vi "VIH Project - Get Effective Group Rule.vi"(7 "Ignore Control Rules (F)":bool, 8 "error in":errorcluster, 10 "Group ID":string, 11 "Project Tree":T1) -> (0 "error out":errorcluster, 2 "Effective Group Rule":T2, 3 "dup Project Tree":T1)   [LabVIEW 2014]
doc: "::: VI Helpeks :::\nCopyright (c) 2000-2026 Konstantin Shifershteyn. All rights reserved."
uses:
  VIH Project Tree Typedef - Tree Refnum.ctl
  _VIH HelpGen.llb/VIH HelpGen Typedef - Cluster - Group Rule.ctl
  _VIH HelpGen.llb/VIH HelpGen Typedef - Enum - Default,Enable,Disable.ctl
  _VIH HelpGen.llb/VIH HelpGen Typedef - Cluster - Group Rule - Source Paths.ctl
  _VIH HelpGen.llb/VIH HelpGen Typedef - Cluster - Group Rule - Target Paths.ctl
  _VIH HelpGen.llb/VIH HelpGen Typedef - Enum - Description Mode.ctl
  _VIH HelpGen.llb/VIH HelpGen Typedef - Cluster - Control Rule.ctl
  _VIH HelpGen.llb/VIH HelpGen Typedef - Cluster - Enum Value Info.ctl
  _VIH HelpGen.llb/VIH HelpGen Typedef - Cluster - Group Rule - Flags.ctl
  VIH Project Tree Typedef - Tree Item Type.ctl
panel:
  # "VI Helpeks\nCopyright (c) 2012-2026 Konstantin Shifershteyn"
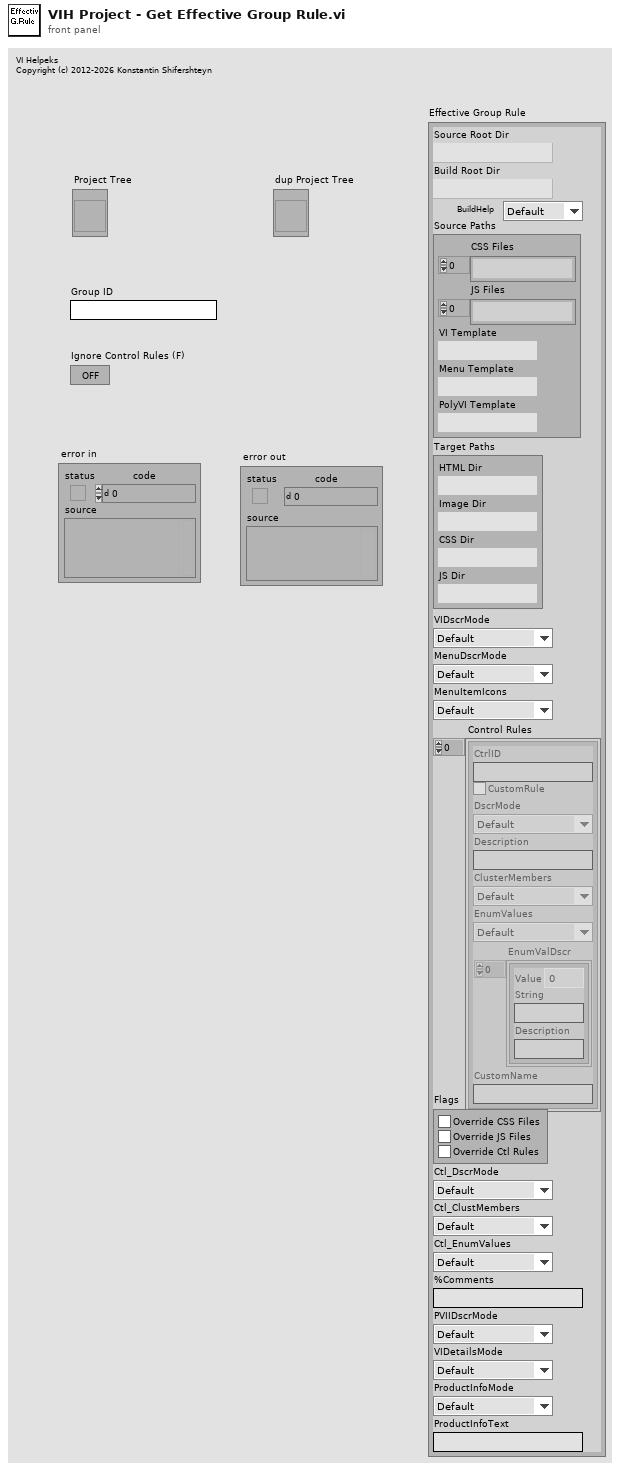
[diagram p1: front panel]
types:
  T1 = typedef "VIH Project Tree Typedef - Tree Refnum.ctl" = refnum<vi>
  T2 = typedef "VIH HelpGen Typedef - Cluster - Group Rule.ctl" = cluster{"Source Root Dir":path, "Build Root Dir":path, "BuildHelp":T3, "Source Paths":T4, "Target Paths":T5, "VIDscrMode":T6, "MenuDscrMode":T6, "MenuItemIcons":T3, "Control Rules":T7[], "Flags":T9, "Ctl_DscrMode":T6, "Ctl_ClustMembers":T3, "Ctl_EnumValues":T3, "%Comments":string, "PVIIDscrMode":T6, "VIDetailsMode":T6, "ProductInfoMode":T3, "ProductInfoText":string}
  T3 = typedef "VIH HelpGen Typedef - Enum - Default,Enable,Disable.ctl" = enum16{"Default", "Enable", "Disable"}
  T4 = typedef "VIH HelpGen Typedef - Cluster - Group Rule - Source Paths.ctl" = cluster{"CSS Files":path[], "JS Files":path[], "VI Template":path, "Menu Template":path, "PolyVI Template":path}
  T5 = typedef "VIH HelpGen Typedef - Cluster - Group Rule - Target Paths.ctl" = cluster{"HTML Dir":path, "Image Dir":path, "CSS Dir":path, "JS Dir":path}
  T6 = typedef "VIH HelpGen Typedef - Enum - Description Mode.ctl" = enum16{"Default", "Description", "Description1", "Description2", "Custom", "None"}
  T7 = typedef "VIH HelpGen Typedef - Cluster - Control Rule.ctl" = cluster{"CtrlID":string, "CustomRule":bool, "DscrMode":T6, "Description":string, "ClusterMembers":T3, "EnumValues":T3, "EnumValDscr":T8[], "CustomName":string}
  T8 = typedef "VIH HelpGen Typedef - Cluster - Enum Value Info.ctl" = cluster{"Value":ext, "String":string, "Description":string}
  T9 = typedef "VIH HelpGen Typedef - Cluster - Group Rule - Flags.ctl" = cluster{"Override CSS Files":bool, "Override JS Files":bool, "Override Ctl Rules":bool}
  T10 = typedef "VIH Project Tree Typedef - Tree Item Type.ctl" = enum32{"<Invalid>", "Project", "Proj Files", "Proj Rules", "File Group", "Rule Group", "Any File", "LV Func", ".mnu", ".mnu (dyn)", ".vi", ".vi (dyn)", ".vit", ".vit (dyn)", ".ctl", ".ctl (dyn)", ".ctt", ".ctt (dyn)", "polyVI", "polyVI (dyn)", "expVI", "expVI (dyn)", "HTML", "PolyVI Inst"}
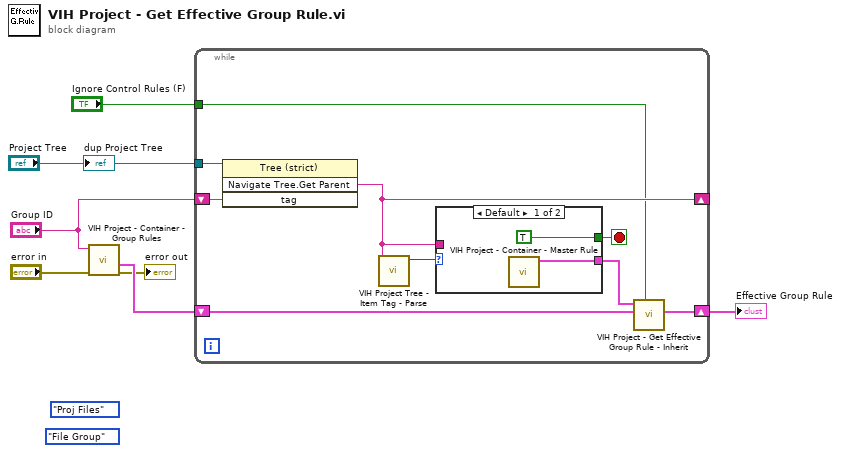
[diagram p0: block diagram]
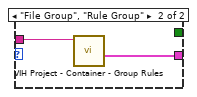
[diagram p2: hidden frame]
diagram:
  (unwired) VIH_Project_Tree_Typedef_-_Tree_Item_Type."File Group" ("Item Type")
  (unwired) VIH_Project_Tree_Typedef_-_Tree_Item_Type."Proj Files" ("Item Type")
  n1 = call "VIH Project - Container - Group Rules.vi"("error in"="error in", "Group ID"="Group ID") -> ("error out"=→"error out":errorcluster, "Group Rule out"=w6:T2)  [unwired: 5 in, 3 out]
  n2 = while {
    tunnel: "Project Tree" -> [w16]
    shift-right: [w11] -> w5
    shift-left: w6 -> [w12]
    shift-right: [w13] -> _
    shift-left: "Group ID" -> [w15]
    tunnel: "Ignore Control Rules (F)" -> [w8]
    stop <- w9 stop-if-true
    n3 = invoke class="Tree (strict)" method="Navigate Tree.Get Parent"(reference=w16, "tag"=w15) -> ("Navigate Tree:Get Parent"=w13:string)  [unwired: 2 in, 3 out]
    n4 = call "VIH Project Tree - Item Tag - Parse.vi"("Tree Item Tag"=w13) -> ("Item Type"=w14:T10)  [unwired: 8 in, 2 out]
    n5 = case shown="Default" w14 {
      tunnel: w13 -> [_ w20]
      tunnel: [w18 w19] -> w10
      tunnel: [TRUE _] -> w9
      frame Default {
        n6 = call "VIH Project - Container - Master Rule.vi"() -> ("Rule out"=w18:T2)  [unwired: 11 in]
      }
      frame "File Group", "Rule Group" {
        n7 = call "VIH Project - Container - Group Rules.vi"("Group ID"=w20) -> ("Group Rule out"=w19:T2)  [unwired: 6 in, 4 out]
      }
    }
    n8 = call "VIH Project - Get Effective Group Rule - Inherit.vi"("Ignore Control Rules (F)"=w8, "Group Rule"=w12, "Parent Group Rule"=w10) -> ("Effective Group Rule"=w11:T2)  [unwired: 8 in]
  }
  "Effective Group Rule" <- w5
  "dup Project Tree" <- "Project Tree"
